vi "Set NodeID Ign.vi"(8 "error in (no error)":errorcluster, 10 "Tester Tx":refnum<vi>, 11 "folder name":string="NonUDT") -> (0 "error out":errorcluster, 3 "NodeIDs":string[](array[string]))   [LabVIEW 2025]
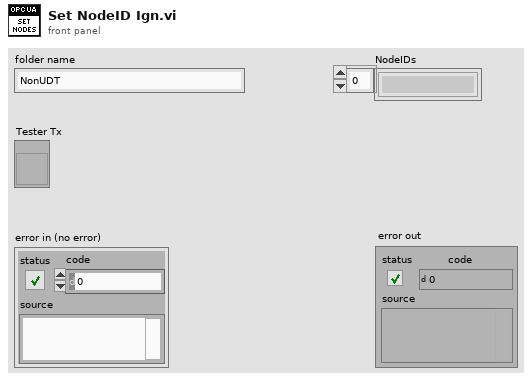
[diagram p1: front panel]
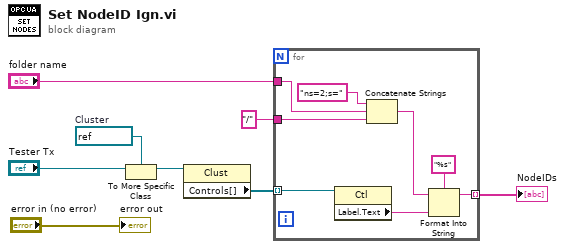
[diagram p0: block diagram]
diagram:
  w5 = refnum<vi> refnum  # Cluster
  n1 = To More Specific Class(target class=w5, reference="Tester Tx") -> (specific class reference=w4:refnum<vi>)  [unwired: 1 in, 1 out]
  n2 = property class="Clust"(reference=w4) -> ("Controls[]"=w6:refnum<vi>[])  [unwired: 1 in, 2 out]
  n3 = for {
    tunnel: w6 -> [w16] mode=indexing
    tunnel: "folder name" -> [w12]
    tunnel: [w13] -> w1 mode=indexing
    tunnel: "/" ("Deliminated Char") -> [w10]
    n4 = property class="Ctl"(reference=w16) -> ("Label.Text"=w15:string)  [unwired: 1 in, 2 out]
    n5 = Concatenate Strings("ns=2;s=" ("format string"), w12, w10) -> (w11:string)
    n6 = Format Into String(format string="%s", initial string=w11, w15) -> (resulting string=w13:string)  [unwired: 1 in, 1 out]
  }
  "NodeIDs" <- w1
  "error out" <- "error in (no error)"
